vi "SMTP Email Send Message.vi"(0 "recipients":string[](array[string]) caption="destinataires", 1 "mail server":string caption="serveur mail", 2 "return address":string caption="adresse de retour", 5 "subject ([No Subject])":string="[Sans objet]" caption="objet ([Sans objet])", 7 "message":string, 11 "error in (no error)":errorcluster caption="entrée d'erreur (pas d'erreur)") -> (4 "invalid recipients":string[](array[string]) caption="destinataires non valides", 15 "error out":errorcluster caption="sortie d'erreur")   [LabVIEW 2022 SP3, in "Copie de NI_SMTPEmail.lvlib"]
doc: "LabVIEW ne supporte plus ce VI. À la place, utilisez le VI Express Envoyer un e-mail.\n\nEnvoie un e-mail texte à une liste de destinataires.\n\nUtilisez le VI SMTP - Envoyer un message (petite taille) pour réduire l'utilisation de mémoire si vous n'avez pas besoin d'envoyer de pièces jointes.\n\n<b>adresse de retour</b> est l'adresse e-mail de l'expéditeur du message. Si vous ne spécifiez pas d'adresse de retour, une chaîne vide est envoyée au serveur. Vous n'êtes pas obligé d'inclure une adresse de retour pour que ce VI fonctionne, mais certains serveurs de messagerie n'acceptent pas les messages si ces informations sont absentes. \n<b>serveur mail</b> est le nom ou l'adresse IP d'un serveur SMTP valide. Si vous passez une chaîne vide à cette entrée, LabVIEW n'accepte pas la connexion réseau et renvoie l'erreur 63. \n<b>destinataires</b> est le tableau de chaînes qui contient les adresses e-mail des destinataires du message. Chaque adresse peut être un élément de tableau séparé. \n<b>objet</b> est la ligne d'objet du message. La valeur par défaut est [Sans objet]. \n<b>message</b> correspond au message textuel de l'e-mail, formaté avec le jeu de caractères système. LabVIEW convertit cette chaîne en format UTF-8 avant d'envoyer l'e-mail. \n<b>entrée d'erreur</b> décrit les conditions d'erreur qui ont lieu avant l'exécution de ce nœud. Cette entrée fournit la fonctionnalité d'entrée d'erreur standard. \n<b>destinataires non valides</b> liste les destinataires rejetés par le serveur mail. \n<b>sortie d'erreur</b> contient des informations sur l'erreur. Cette sortie fournit la fonctionnalité de sortie d'erreur standard."
uses:
  Copie de NI_SMTPEmail.lvlib
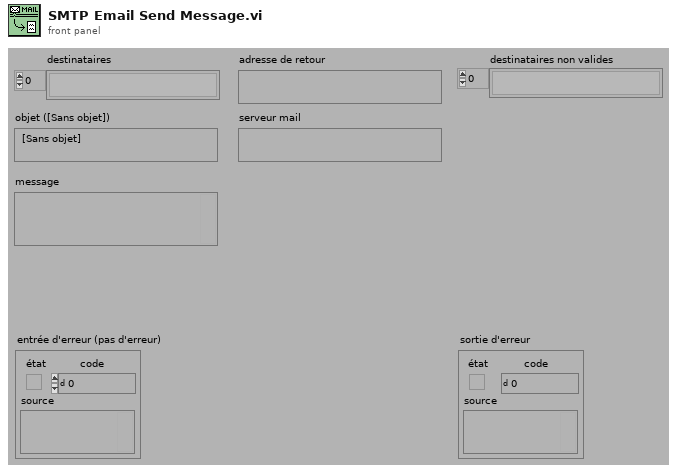
[diagram p1: front panel]
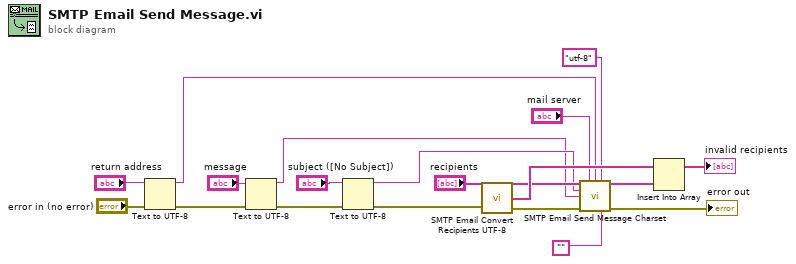
[diagram p0: block diagram]
diagram:
  n1 = Text to UTF-8(8:"error in (no error)", 11:"return address") -> (0:w14:errorcluster, 3:w5:string)  [unwired: 1 in]
  n2 = Text to UTF-8(8:w14, 11:"message") -> (0:w15:errorcluster, 3:w6:string)  [unwired: 1 in]
  n3 = Text to UTF-8(8:w15, 11:"subject ([No Subject])") -> (0:w12:errorcluster, 3:w7:string)  [unwired: 1 in]
  n4 = call "SMTP Email Convert Recipients UTF-8.vi"("recipients"="recipients", "error in"=w12) -> ("convertible recipients"=w8:string[], "unconvertible recipients"=w10:string[], "error out"=w2:errorcluster)
  n5 = call "SMTP Email Send Message Charset.vi"("recipients"=w8, "mail server"="mail server", "return address"=w5, "character set (us-ascii)"="utf-8", "subject ([No Subject])"=w7, "message"=w6, "error in (no error)"=w2, "translit"="") -> ("invalid recipients"=w11:string[], "error out"=→"error out":errorcluster)  [unwired: 6 in]
  n6 = Insert Into Array(array=w10, new element=w11) -> (→"invalid recipients":string[])  [unwired: 1 in]
